vi "FX_Open.vi"(9 "error in (no error)":errorcluster, 10 "Serial (COM)?":bool, 11 "Resource":refnum<visa-resource-name>) -> (2 "error out":errorcluster, 3 "VISA out":refnum<visa-resource-name>)   [LabVIEW 2018]
doc: "Use this template to build a VI to use as a subVI."
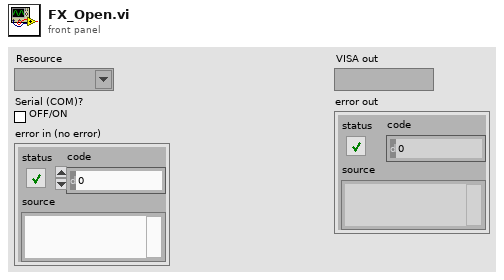
[diagram p1: front panel]
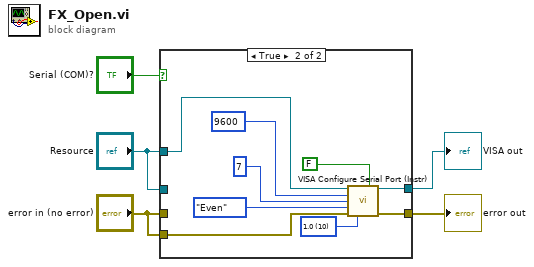
[diagram p0: block diagram]
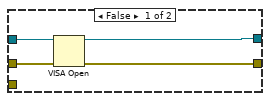
[diagram p2: hidden frame]
diagram:
  n1 = case shown="True" "Serial (COM)?" {
    tunnel: "Resource" -> [w9 _]
    tunnel: "error in (no error)" -> [w8 _]
    tunnel: "Resource" -> [_ w18]
    tunnel: "error in (no error)" -> [_ w17]
    tunnel: [w7 w11] -> w2
    tunnel: [w6 w10] -> w1
    frame False {
      n2 = VISA Open(error in (no error)=w8, VISA resource name=w9) -> (VISA resource name=w7:refnum<visa-resource-name>, error out=w6:errorcluster)  [unwired: 3 in]
    }
    frame True {
      w13 = u16 10 items=["1.0"=10, "1.5"=15, "2.0"=20] ("stop bits (10: 1 bit)")
      n3 = call <vilib>:"VISA Configure Serial Port (Instr).vi"("VISA resource name"=w18, "Enable Termination\nChar (T)"=FALSE, "baud rate (9600)"=u32 9600, "data bits (8)"=u16 7, "parity (0:none)"=enum16{"None", "Odd", "Even", "Mark", "Space"}."Even", "error in (no error)"=w17, "stop bits (10: 1 bit)"=w13) -> ("VISA resource name out"=w11:refnum<visa-resource-name>, "error out"=w10:errorcluster)  [unwired: 7 in]
    }
  }
  "VISA out" <- w2
  "error out" <- w1
